vi "libssh2_sftp_seek64.vi"(8 "error in (no error)":errorcluster, 10 "offset":u64, 11 "sftp handle":T1) -> (0 "error out":errorcluster)   [LabVIEW 2017, in "libssh2.lvlib"]
doc: "Set the file position of a file handle."
uses:
  libssh2.lvlib
  SFTP Handle Refnum.ctl
  Acquire SFTP.vi
  Release SFTP.vi
  Acquire Session.vi
  Release Session.vi
  Not An SFTP Handle Refnum.vi
  <vilib>/Utility/error.llb/Error Cluster From Error Code.vi
  Global Settings.vi
  Read SFTP Handle Refnum.vi
  Read SFTP Refnum.vi
  Read Session Refnum.vi
  <vilib>/Utility/semaphor.llb/Acquire Semaphore.vi
  <vilib>/Utility/semaphor.llb/Release Semaphore.vi
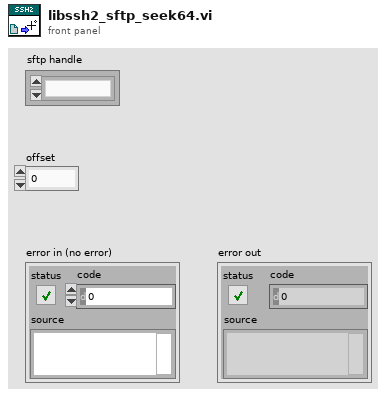
[diagram p1: front panel]
types:
  T1 = typedef "libssh2.lvlib/SFTP Handle Refnum.ctl" = refnum<k1>
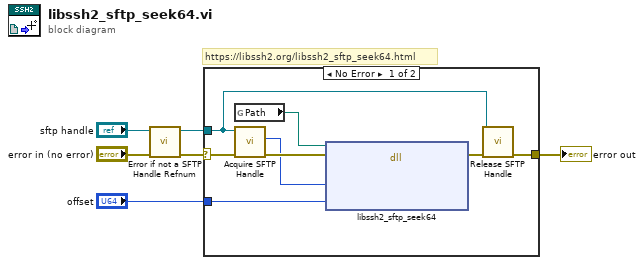
[diagram p0: block diagram]
diagram:
  # "https://libssh2.org/libssh2_sftp_seek64.html"
  n1 = call "Error if not a SFTP Handle Refnum.vi"("error in (no error)"="error in (no error)", "sftp handle"="sftp handle") -> ("error out"=w5:errorcluster, "sftp handle out"=w4:T1)  [unwired: 8 in]
  n2 = case shown="No Error" w5 {
    selector: w5 -> [w13 w15]
    tunnel: w4 -> [w7 _]
    tunnel: [w8 w15] -> w3
    tunnel: "offset" -> [w9 _]
    frame No Error {
      n3 = global read "Global Settings.vi" "Path"() -> (w14:path)
      n4 = call "Acquire SFTP Handle.vi"("error in (no error)"=w13, "sftp handle"=w7) -> ("error out"=w12:errorcluster, "LIBSSH2_SFTP_HANDLE*"=w11:u64)  [unwired: 8 in]
      n5 = dll-call lib="?" fn="libssh2_sftp_seek64"(path in=w14, error in=w12, "handle"=w11, "offset"=w9) -> (error out=w10:errorcluster)  [unwired: 4 in, 1 out]
      n6 = call "Release SFTP Handle.vi"("error in (no error)"=w10, "sftp handle"=w7) -> ("error out"=w8:errorcluster)  [unwired: 9 in]
    }
    frame Error {
    }
  }
  "error out" <- w3
